vi "FuncVI-scanstr.vi"(5 "InstanceRef":T2, 9 "arg list":T1[](array[typedef]) {"num" format="%.2f"}) -> (0 "error out":bool, 3 "result":T1 {"num" format="%.2f"})   [LabVIEW 2021]
doc: "::: CalcExpress Toolkit :::\nCopyright (c) 2000-2026 Konstantin Shifershteyn. All rights reserved."
uses:
  cetypes.llb/CalcExpress Function Argument Info.ctl
  cetypes.llb/CalcExpress Instance RefNum.ctl
panel:
  in  "max arg num":i32=3
  in  "min arg num":i32=1
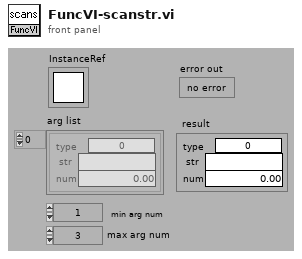
[diagram p1: front panel]
types:
  T1 = typedef "CalcExpress Function Argument Info.ctl" = cluster{"type":u32, "str":string, "num":dbl}
  T2 = typedef "CalcExpress Instance RefNum.ctl" = refnum<k1>
  T3 = enum32{"String", "DBL Number", "identifier", "1D Array of DBL", "2D Array of DBL", "CDB Number", "1D Array of CDB", "2D Array of CDB", "1D Array of String", "2D Array of String", "Unknown data type"}
  T4 = cluster{"index":i32, "data type":enum32{"String", "DBL Number", "identifier", "1D Array of DBL", "2D Array of DBL", "CDB Number", "1D Array of CDB", "2D Array of CDB", "1D Array of String", "2D Array of String", "Unknown data type"}, "default num":dbl, "default str":string}[]
  T5 = cluster{"data type":enum32{"String", "DBL Number", "identifier", "1D Array of DBL", "2D Array of DBL", "CDB Number", "1D Array of CDB", "2D Array of CDB", "1D Array of String", "2D Array of String", "Unknown data type"}, string, dbl}
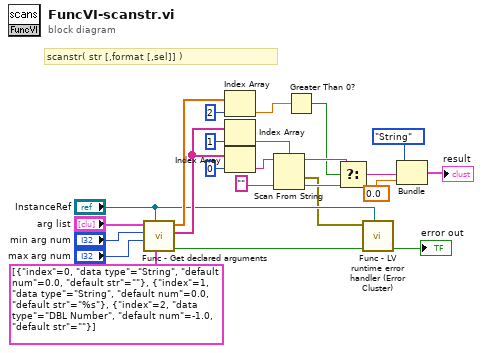
[diagram p0: block diagram]
diagram:
  # "scanstr( str [,format [,sel]] )"
  n1 = call "Func - Get declared arguments.vi"("arg descriptors"=T4 [{"index"=0, "data type"=enum."String", "default num"=0.0, "default str"=""}, {"index"=1, "data type"=enum."String", "default num"=0.0, "default str"="%s"}, {"index"=2, "data type"=enum."DBL Number", "default num"=-1.0, "default str"=""}] ("args descriptors"), "InstanceRef"="InstanceRef", "max arg num"="max arg num", "min arg num"="min arg num", "arg list"="arg list") -> ("error out"=w4:bool, "str list"=w20:string[], "num list"=w15:dbl[])  [unwired: 3 in, 1 out]
  n2 = Index Array(array=w15, index=2) -> (element=w7:dbl)
  n3 = Index Array(array=w20, index=1) -> (element=w19:string)
  n4 = Index Array(array=w20, index=0) -> (element=w18:string)
  n5 = Scan From String(format string=w19, input string=w18, default 1="") -> (remaining string=w14:string, error out=w2:errorcluster, output 1=w13:string)  [unwired: 2 in, 1 out]
  n6 = Greater Than 0?(x=w7) -> (x > 0?=w12:bool)
  n7 = Select(t=w14, s=w12, f=w13) -> (s? t:f=w11:string)
  n8 = call "Func - LV runtime error handler (Error Cluster).vi"("InstanceRef"="InstanceRef", "error in"=w4, "LabVIEW error"=w2) -> ("error out"=→"error out":bool)  [unwired: 3 in, 3 out]
  n9 = Bundle("data type"=T3."String", w11, 0.0) -> (→"result":T5)  [unwired: 1 in]
